vi "Correct_Disconnection_101_and_11_Point-1.vi"(4 "error IN":errorcluster, 7 "[IN] Still connected\ntracks in group":T2) -> (0 "error OUT":errorcluster, 3 "[OUT] Clusters for Re\nconstructed Tracks":T1)   [LabVIEW 2017]
doc: "Correction of the mistake when an origin and an elongation of tracks become disconnected"
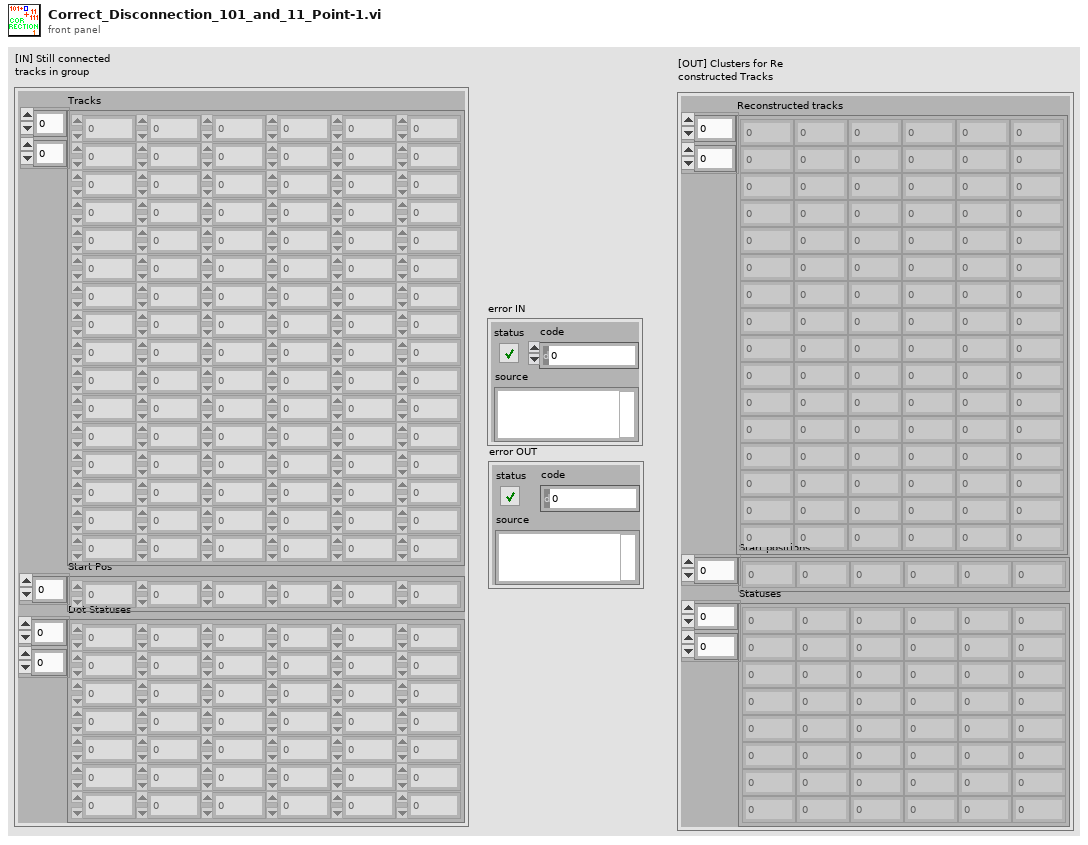
[diagram p1: front panel]
types:
  T1 = cluster{"Reconstructed tracks":dbl[][], "Start positions":i32[], "Statuses":i16[][]}
  T2 = cluster{"Tracks":dbl[][], "Start Pos":i32[], "Dot Statuses":i16[][]}
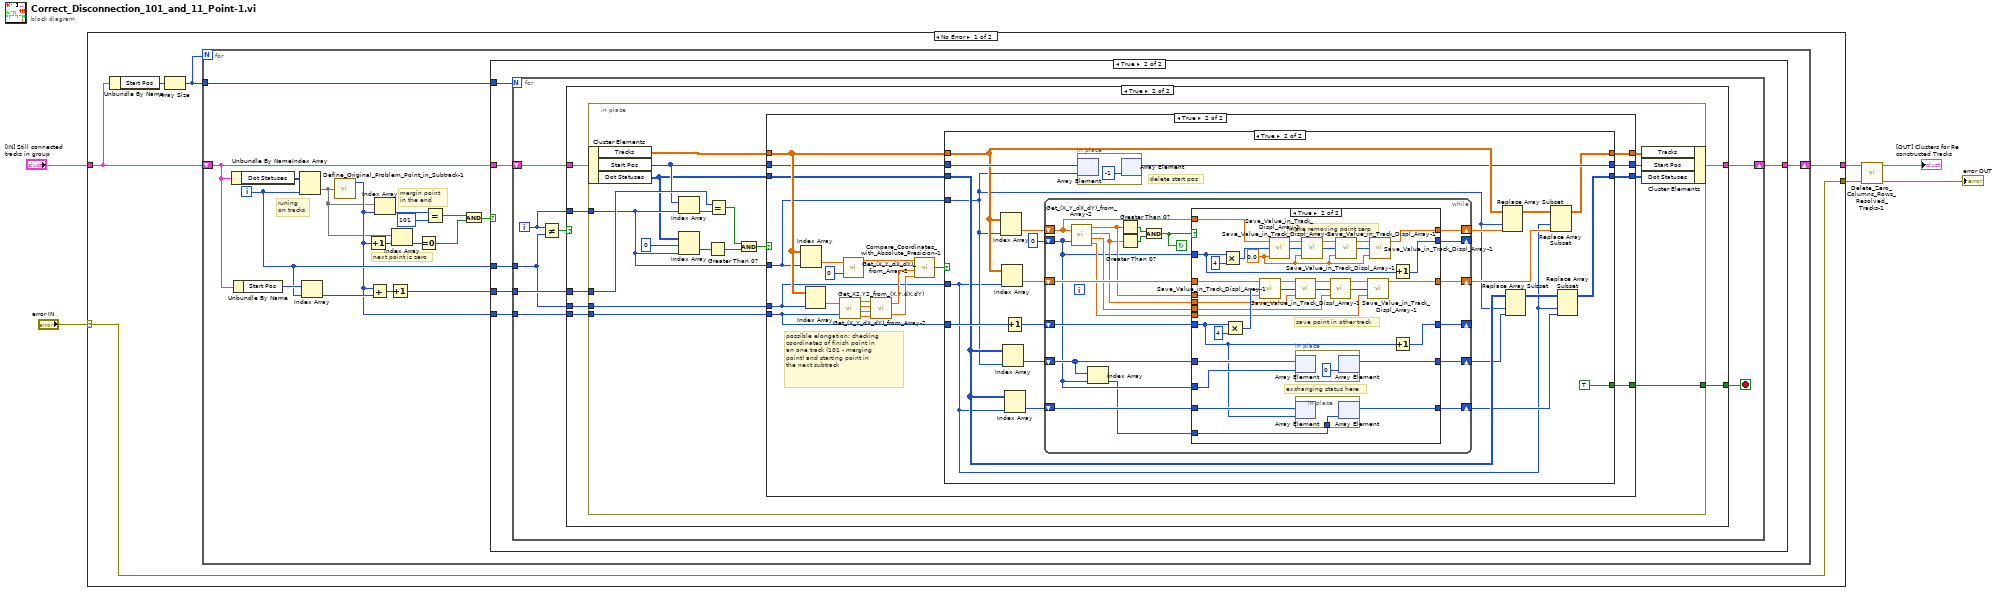
[diagram p0: block diagram]
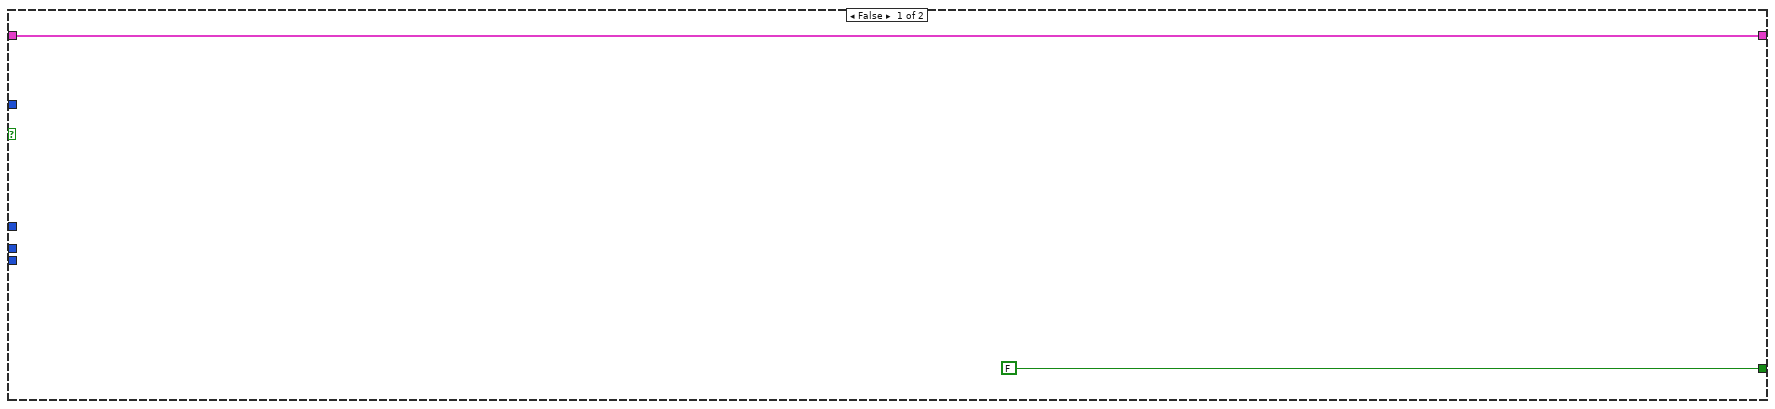
[diagram p3: hidden frame]
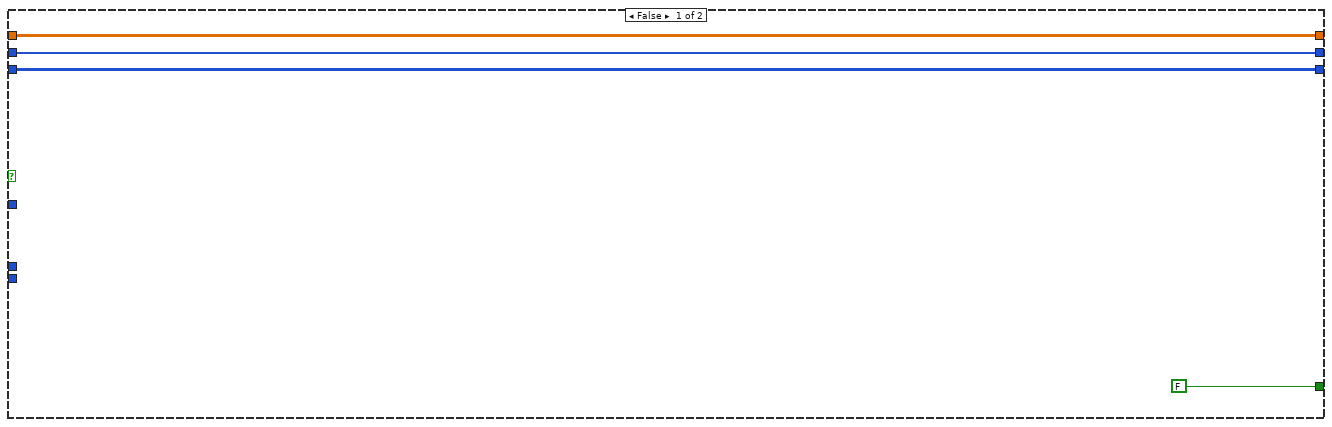
[diagram p4: hidden frame]
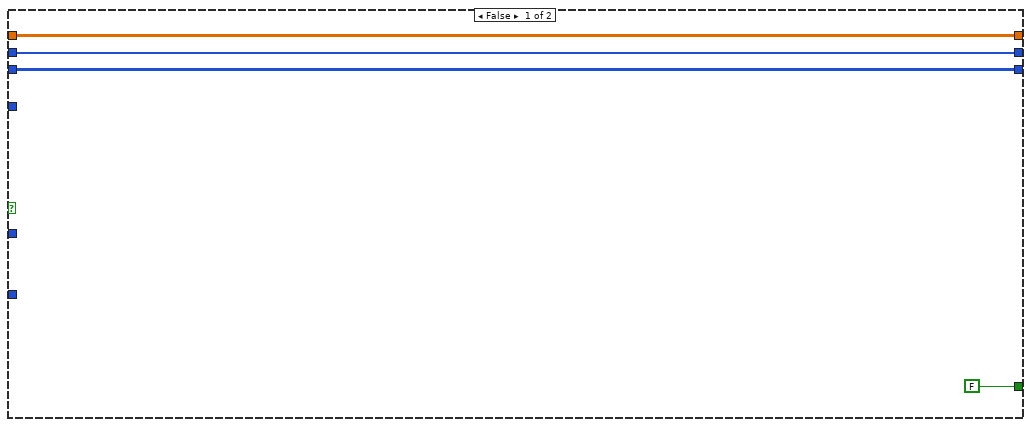
[diagram p5: hidden frame]
diagram:
  n1 = case shown="No Error" "error IN" {
    selector: "error IN" -> [w8 w187]
    tunnel: "[IN] Still connected\ntracks in group" -> [w10 w188]
    tunnel: [w8 w187] -> w3
    tunnel: [w7 w188] -> w4
    frame No Error {
      n2 = Unbundle By Name(w10) -> ("Start Pos"=w11:i32[])
      n3 = Array Size(array=w11) -> (size(s)=w9:i32)
      n4 = for {
        N: w9 -> [_]
        shift-right: [w17] -> w7
        shift-left: w10 -> [w24]
        tunnel: w9 -> [w29]
        i -> [w22]
        # "mergin point \nin the end"
        # "runing \non tracks"
        # "next point is zero"
        n5 = Unbundle By Name(w24) -> ("Dot Statuses"=w25:i16[][])
        n6 = Unbundle By Name(w24) -> ("Start Pos"=w23:i32[])
        n7 = Index Array(array=w25, index (col)=w22) -> (element=w15:i16[])  [unwired: 1 in]
        n8 = Index Array(array=w23, index=w22) -> (element=w21:i32)
        n9 = call "Define_Original_Problem_Point_in_Subtrack-1.vi"("[IN] Statuses"=w15) -> ("[OUT] Index of Problem Point\nin Subtrack (Original)"=w18:i32)  [unwired: 3 in, 1 out]
        n10 = Increment(x=w18) -> (x+1=w27:i32)
        n11 = Add(x=w18, y=w21) -> (x+y=w20:i32)
        n12 = Index Array(array=w15, index=w18) -> (element=w16:i16)
        n13 = Increment(x=w20) -> (x+1=w19:i32)
        n14 = Index Array(array=w15, index=w27) -> (element=w28:i16)
        n15 = Equal To 0?(x=w28) -> (x = 0?=w13:bool)
        n16 = Equal?(x=w16, y=i16 101) -> (x = y?=w14:bool)
        n17 = And(x=w14, y=w13) -> (x .and. y?=w12:bool)
        n18 = case shown="True" w12 {
          tunnel: w29 -> [_ w36]
          tunnel: w24 -> [w30 w35]
          tunnel: w22 -> [_ w34]
          tunnel: w19 -> [_ w33]
          tunnel: w18 -> [_ w32]
          tunnel: [w30 w31] -> w17
          frame False {
          }
          frame True {
            n19 = for {
              N: w36 -> [_]
              shift-right: [w38] -> w31
              shift-left: w35 -> [w43]
              tunnel: w34 -> [w40]
              tunnel: w33 -> [w41]
              tunnel: w32 -> [w39]
              i -> [w42]
              stop <- w37 stop-if-true
              n20 = Not Equal?(x=w42, y=w40) -> (x != y?=w44:bool)
              n21 = case shown="True" w44 {
                tunnel: w43 -> [w46 w53]
                tunnel: w42 -> [_ w52]
                tunnel: w41 -> [_ w51]
                tunnel: w40 -> [_ w50]
                tunnel: w39 -> [_ w49]
                tunnel: [w46 w48] -> w38
                tunnel: [FALSE w47] -> w37
                frame False {
                }
                frame True {
                  n22 = in-place {
                    in-place-border: w52 -> [w63]
                    in-place-border: w51 -> [w66]
                    in-place-border: w50 -> [w62]
                    in-place-border: w49 -> [w61]
                    in-place-border: [w55] -> w47
                    n23 = in-place-cluster #1(w53) -> ("Tracks"=w64:dbl[][], "Start Pos"=w60:i32[], "Dot Statuses"=w59:i16[][])
                    n24 = Index Array(array=w60, index=w63) -> (element=w67:i32)
                    n25 = Index Array(array=w59, index (row)=0 ("disabled index (row)"), index (col)=w63) -> (element=w68:i16)
                    n26 = Greater Than 0?(x=w68) -> (x > 0?=w54:bool)
                    n27 = Equal?(x=w66, y=w67) -> (x = y?=w69:bool)
                    n28 = And(x=w69, y=w54) -> (x .and. y?=w65:bool)
                    n29 = case shown="True" w65 {
                      tunnel: w64 -> [w74 w84]
                      tunnel: w63 -> [_ w80]
                      tunnel: w62 -> [_ w79]
                      tunnel: w61 -> [_ w81]
                      tunnel: w60 -> [w73 w83]
                      tunnel: w59 -> [w72 w82]
                      tunnel: [w73 w78] -> w58
                      tunnel: [w74 w77] -> w57
                      tunnel: [w72 w76] -> w56
                      tunnel: [FALSE w75] -> w55
                      frame False {
                      }
                      frame True {
                        # "possible elongation: checking \ncoordinates of finish point in \nan one track (101 - merging\npoint) and starting point in \nthe next subtrack"
                        n30 = Index Array(array=w84, index (col)=w80) -> (element=w96:dbl[])  [unwired: 1 in]
                        n31 = Index Array(array=w84, index (col)=w79) -> (element=w94:dbl[])  [unwired: 1 in]
                        n32 = call "Get_(X_Y_dX_dY)_from_Array-2.vi"("(X,Y,dX,dY)"=w94, "Index of Displacement"=w81) -> ("X"=w93:dbl, "Y"=w92:dbl, "dX"=w91:dbl, "dY"=w90:dbl)
                        n33 = call "Get_(X_Y_dX_dY)_from_Array-2.vi"("(X,Y,dX,dY)"=w96, "Index of Displacement"=0 ("disabled index (row)")) -> ("X"=w89:dbl, "Y"=w88:dbl)  [unwired: 2 out]
                        n34 = call "Get_X2,Y2_from_(X,Y,dX,dY).vi"("dY"=w90, "dX"=w91, "Y1"=w92, "X1"=w93) -> ("Y2 = (Y1+dY)"=w86:dbl, "X2 = (X1+dX)"=w87:dbl)
                        n35 = call "Compare_Coordinates_with_Absolute_Presicion-1.vi"("X 1"=w89, "Y 1"=w88, "X 2"=w87, "Y 2"=w86) -> ("[OUT] Same coordinates?"=w85:bool)  [unwired: 1 in]
                        n36 = case shown="True" w85 {
                          tunnel: w84 -> [w100 w114]
                          tunnel: w83 -> [w99 w122]
                          tunnel: w82 -> [w98 w110]
                          tunnel: w81 -> [_ w120]
                          tunnel: w80 -> [_ w108]
                          tunnel: w79 -> [_ w105]
                          tunnel: [w99 w104] -> w78
                          tunnel: [w100 w103] -> w77
                          tunnel: [w98 w102] -> w76
                          tunnel: [FALSE TRUE] -> w75
                          frame False {
                          }
                          frame True {
                            # "delete start pos"
                            n37 = Index Array(array=w114, index (col)=w108) -> (element=w121:dbl[])  [unwired: 1 in]
                            n38 = Index Array(array=w114, index (col)=w105) -> (element=w119:dbl[])  [unwired: 1 in]
                            n39 = Index Array(array=w110, index (col)=w108) -> (element=w116:i16[])  [unwired: 1 in]
                            n40 = Increment(x=w120) -> (x+1=w117:i32)
                            n41 = Index Array(array=w110, index (col)=w105) -> (element=w115:i16[])  [unwired: 1 in]
                            n42 = while {
                              shift-right: [w132] -> w113
                              shift-left: w121 -> [w139]
                              shift-right: [w130] -> w111
                              shift-left: w119 -> [w138]
                              shift-right: [w131] -> _
                              shift-left: 0 -> [w127]
                              shift-right: [w129] -> _
                              shift-left: w117 -> [w137]
                              shift-right: [w126] -> w109
                              shift-left: w116 -> [w128]
                              shift-right: [w123] -> w106
                              shift-left: w115 -> [w125]
                              stop <- w140 continue-if-true
                              n43 = call "Get_(X_Y_dX_dY)_from_Array-2.vi"("(X,Y,dX,dY)"=w139, "Index of Displacement"=w127) -> ("X"=w136:dbl, "Y"=w135:dbl, "dX"=w134:dbl, "dY"=w133:dbl)
                              n44 = Index Array(array=w128, index=w127) -> (element=w124:i16)
                              n45 = Greater Than 0?(x=w136) -> (x > 0?=w142:bool)
                              n46 = Greater Than 0?(x=w135) -> (x > 0?=w141:bool)
                              n47 = And(x=w142, y=w141) -> (x .and. y?=w140:bool)
                              n48 = case shown="True" w140 {
                                tunnel: w139 -> [w148 w174]
                                tunnel: w127 -> [w147 w160]
                                tunnel: w138 -> [w146 w172]
                                tunnel: w137 -> [w145 w151]
                                tunnel: w136 -> [_ w170]
                                tunnel: w135 -> [_ w167]
                                tunnel: w134 -> [_ w164]
                                tunnel: w133 -> [_ w161]
                                tunnel: [w148 w159] -> w132
                                tunnel: [w147 w158] -> w131
                                tunnel: [w146 w157] -> w130
                                tunnel: [w145 w156] -> w129
                                tunnel: w128 -> [w144 w155]
                                tunnel: w127 -> [_ w154]
                                tunnel: [w144 w153] -> w126
                                tunnel: w125 -> [w143 w152]
                                tunnel: w124 -> [_ w150]
                                tunnel: [w143 w149] -> w123
                                frame False {
                                }
                                frame True {
                                w183 = 0.0 ("[IN] Value")
                                # "exchanging status here"
                                # "make removing point zero"
                                # "save point in other track"
                                n49 = Multiply(x=w160, y=4) -> (x*y=w175:i32)
                                n50 = Multiply(x=w151, y=4) -> (x*y=w171:i32)
                                n51 = call "Save_Value_in_Track_Displ_Array-1.vi"("[IN] Value"=w170, "[IN] Index"=w171, "[IN] Empty tracks\nfor points saving"=w172) -> ("[OUT] Index ++"=w168:i32, "[OUT Track with saved value"=w169:dbl[])  [unwired: 1 in]
                                n52 = call "Save_Value_in_Track_Displ_Array-1.vi"("[IN] Value"=w183, "[IN] Index"=w175, "[IN] Empty tracks\nfor points saving"=w174) -> ("[OUT] Index ++"=w178:i32, "[OUT Track with saved value"=w177:dbl[])  [unwired: 1 in]
                                n53 = call "Save_Value_in_Track_Displ_Array-1.vi"("[IN] Value"=w167, "[IN] Index"=w168, "[IN] Empty tracks\nfor points saving"=w169) -> ("[OUT] Index ++"=w165:i32, "[OUT Track with saved value"=w166:dbl[])  [unwired: 1 in]
                                n54 = in-place {
                                n55 = in-place-array #2(w155, w154) -> ()  [unwired: 1 out]
                                n56 = in-place-array #2(i16 0 ("element")) -> (w153:i16[])  [unwired: 1 out]
                                }
                                n57 = in-place {
                                in-place-border: w150 -> [w184]
                                n58 = in-place-array #3(w152, w151) -> ()  [unwired: 1 out]
                                n59 = in-place-array #3(w184) -> (w149:i16[])  [unwired: 1 out]
                                }
                                n60 = call "Save_Value_in_Track_Displ_Array-1.vi"("[IN] Value"=w183, "[IN] Index"=w178, "[IN] Empty tracks\nfor points saving"=w177) -> ("[OUT] Index ++"=w180:i32, "[OUT Track with saved value"=w179:dbl[])  [unwired: 1 in]
                                n61 = call "Save_Value_in_Track_Displ_Array-1.vi"("[IN] Value"=w164, "[IN] Index"=w165, "[IN] Empty tracks\nfor points saving"=w166) -> ("[OUT] Index ++"=w162:i32, "[OUT Track with saved value"=w163:dbl[])  [unwired: 1 in]
                                n62 = call "Save_Value_in_Track_Displ_Array-1.vi"("[IN] Value"=w183, "[IN] Index"=w180, "[IN] Empty tracks\nfor points saving"=w179) -> ("[OUT] Index ++"=w182:i32, "[OUT Track with saved value"=w181:dbl[])  [unwired: 1 in]
                                n63 = call "Save_Value_in_Track_Displ_Array-1.vi"("[IN] Value"=w161, "[IN] Index"=w162, "[IN] Empty tracks\nfor points saving"=w163) -> ("[OUT Track with saved value"=w157:dbl[])  [unwired: 1 in, 1 out]
                                n64 = call "Save_Value_in_Track_Displ_Array-1.vi"("[IN] Value"=w183, "[IN] Index"=w182, "[IN] Empty tracks\nfor points saving"=w181) -> ("[OUT Track with saved value"=w159:dbl[])  [unwired: 1 in, 1 out]
                                n65 = Increment(x=w151) -> (x+1=w156:i32)
                                n66 = Increment(x=w160) -> (x+1=w158:i32)
                                }
                              }
                            }
                            n67 = in-place {
                              n68 = in-place-array #4(w122, w108) -> ()  [unwired: 1 out]
                              n69 = in-place-array #4(-1) -> (w104:i32[])  [unwired: 1 out]
                            }
                            n70 = Replace Array Subset(array=w114, new element=w113, index (col)=w108) -> (w112:dbl[][])  [unwired: 1 in]
                            n71 = Replace Array Subset(array=w110, new element=w109, index (col)=w108) -> (w107:i16[][])  [unwired: 1 in]
                            n72 = Replace Array Subset(array=w112, new element=w111, index (col)=w105) -> (w103:dbl[][])  [unwired: 1 in]
                            n73 = Replace Array Subset(array=w107, new element=w106, index (col)=w105) -> (w102:i16[][])  [unwired: 1 in]
                          }
                        }
                      }
                    }
                    n74 = in-place-cluster #1("Tracks"=w57, "Start Pos"=w58, "Dot Statuses"=w56) -> (w48:T2)
                  }
                }
              }
            }
          }
        }
      }
    }
    frame Error {
    }
  }
  n75 = call "Delete_Zero_Columns_Rows_Resolved_Tracks-1.vi"("error IN"=w3, "[IN] Clusters for Re\nconstructed Tracks"=w4) -> ("error OUT"=→"error OUT":errorcluster, "[OUT] Clusters for Re\nconstructed Tracks"=→"[OUT] Clusters for Re\nconstructed Tracks":T1)  [unwired: 4 in]
